vi "test broken tool message.vi"(8 "error in (no error)":errorcluster) -> (0 "error out":errorcluster, 3 "body":string)   [LabVIEW 2020, in "MCP Server tests.lvlib"]
doc: "Calling a tool whose VI is not executable is a tool execution error: a normal result with isError true and one text item that says the VI is not executable. No JSON-RPC error, no LabVIEW call chain."
uses:
  MCP Server tests.lvlib
  <vilib>/JDP Science/JSONtext/Next JSON Value.vi
  <vilib>/JDP Science/JSONtext/String Subset.vi
  <vilib>/JDP Science/JSONtext/Parsing/Advance past next JSON Value (inlined COPY).vi
  <vilib>/JDP Science/JSONtext/Parsing/Advance past whitespace.vi
  <vilib>/JDP Science/JSONtext/Parsing/Advance past String.vi
  <vilib>/JDP Science/JSONtext/Parsing/Advance past Number.vi
  <vilib>/JDP Science/JSONtext/Parsing/Advance past Line Ending.vi
  <vilib>/JDP Science/JSONtext/Parsing/Parse Full Path or Item Name.vi
  <vilib>/JDP Science/JSONtext/Parsing/Advance past Array.vi
  <vilib>/JDP Science/JSONtext/Parsing/Advance past Object.vi
  <vilib>/JDP Science/JSONtext/support/Error Cluster From Code.vi
  <vilib>/JDP Science/JSONtext/Offset/Find Item Locations by Path.vi
  <vilib>/addons/_JKI Toolkits/Caraya/classes/Test/Test.lvclass
  <vilib>/JDP Science/JSONtext/JSONtext.lvlib
  <vilib>/addons/_JKI Toolkits/Caraya/classes/Assert/Assert.lvclass
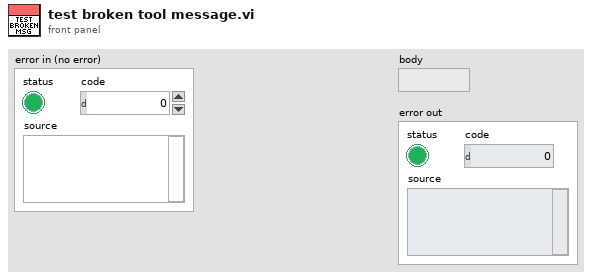
[diagram p1: front panel]
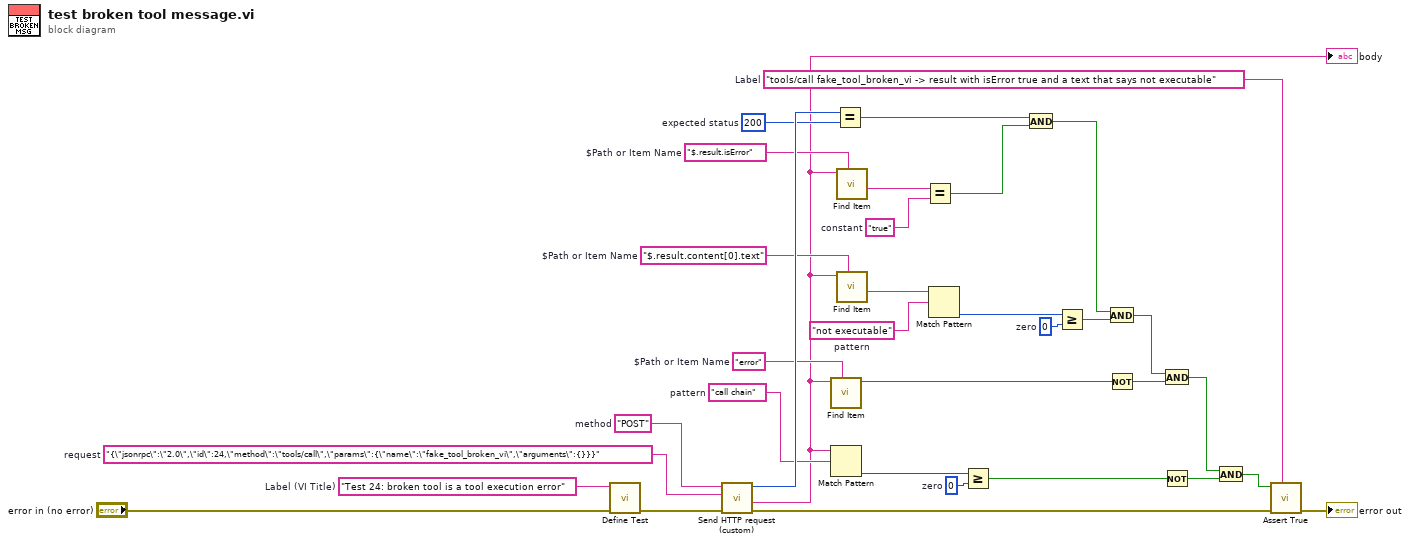
[diagram p0: block diagram]
diagram:
  w3 = "tools/call fake_tool_broken_vi -> result with isError true and a text that says not executable"  # Label
  w15 = 0  # zero
  w17 = "call chain"  # pattern
  w19 = 0  # zero
  w21 = "not executable"  # pattern
  w23 = "true"  # constant
  w25 = "error"  # $Path or Item Name
  w26 = "$.result.content[0].text"  # $Path or Item Name
  w27 = "$.result.isError"  # $Path or Item Name
  w28 = 200  # expected status
  w31 = "{\"jsonrpc\":\"2.0\",\"id\":24,\"method\":\"tools/call\",\"params\":{\"name\":\"fake_tool_broken_vi\",\"arguments\":{}}}"  # request
  w32 = "POST"  # method
  w34 = "Test 24: broken tool is a tool execution error"  # Label (VI Title)
  n1 = call <vilib>:"Define Test.vi"("error in (no error)"="error in (no error)", "Label (VI Title)"=w34) -> ("error out"=w30:errorcluster)  [unwired: 8 in, 1 out]
  n2 = call "Send HTTP request (custom).vi"("error in (no error)"=w30, "request"=w31, "method"=w32) -> ("error out"=w4:errorcluster, "response"=w2:string, "status code"=w29:i32)  [unwired: 5 in, 1 out]
  "body" <- w2
  n3 = call <vilib>:"Find Item.vi"("$Path or Item Name"=w25, "JSON"=w2) -> ("Found"=w18:bool)  [unwired: 6 in, 3 out]
  n4 = Match Pattern(string=w2, regular expression=w17) -> (offset past match=w16:i32)  [unwired: 1 in, 3 out]
  n5 = Equal?(x=w29, y=w28) -> (x = y?=w13:bool)
  n6 = call <vilib>:"Find Item.vi"("$Path or Item Name"=w27, "JSON"=w2) -> ("<JSON>"=w24:string)  [unwired: 6 in, 3 out]
  n7 = call <vilib>:"Find Item.vi"("$Path or Item Name"=w26, "JSON"=w2) -> ("<JSON>"=w22:string)  [unwired: 6 in, 3 out]
  n8 = Equal?(x=w24, y=w23) -> (x = y?=w12:bool)
  n9 = Match Pattern(string=w22, regular expression=w21) -> (offset past match=w20:i32)  [unwired: 1 in, 3 out]
  n10 = Greater Or Equal?(x=w16, y=w15) -> (x >= y?=w14:bool)
  n11 = And(x=w13, y=w12) -> (x .and. y?=w11:bool)
  n12 = Greater Or Equal?(x=w20, y=w19) -> (x >= y?=w10:bool)
  n13 = And(x=w11, y=w10) -> (x .and. y?=w9:bool)
  n14 = Not(x=w18) -> (.not. x?=w8:bool)
  n15 = And(x=w9, y=w8) -> (x .and. y?=w7:bool)
  n16 = Not(x=w14) -> (.not. x?=w6:bool)
  n17 = And(x=w7, y=w6) -> (x .and. y?=w5:bool)
  n18 = call <vilib>:"Assert True.vi"("Label"=w3, "error in (no error)"=w4, "True?"=w5) -> ("error out"=→"error out":errorcluster)  [unwired: 7 in, 1 out]
